vi "Get Python Version from Venv.vi"(8 "error in":errorcluster, 11 "venv":path) -> (0 "error out":errorcluster, 3 "Python Version":string)   [LabVIEW 2026]
doc: "Gets the Python version from a virtual-environment root path. Validates the input path and allowed characters, verifies that the expected Python executable exists, runs the interpreter with --version, and returns the parsed major.minor.patch version string. Returns an error if the venv path is invalid or the Python executable is missing."
uses:
  <vilib>/regexp/Match Regular Expression.xnode
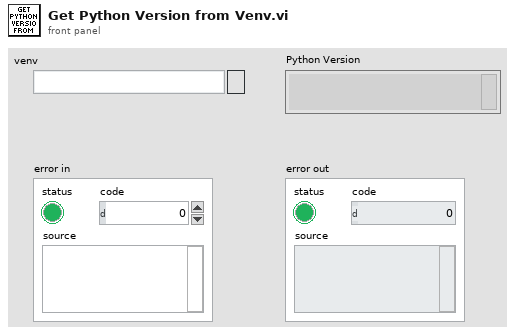
[diagram p1: front panel]
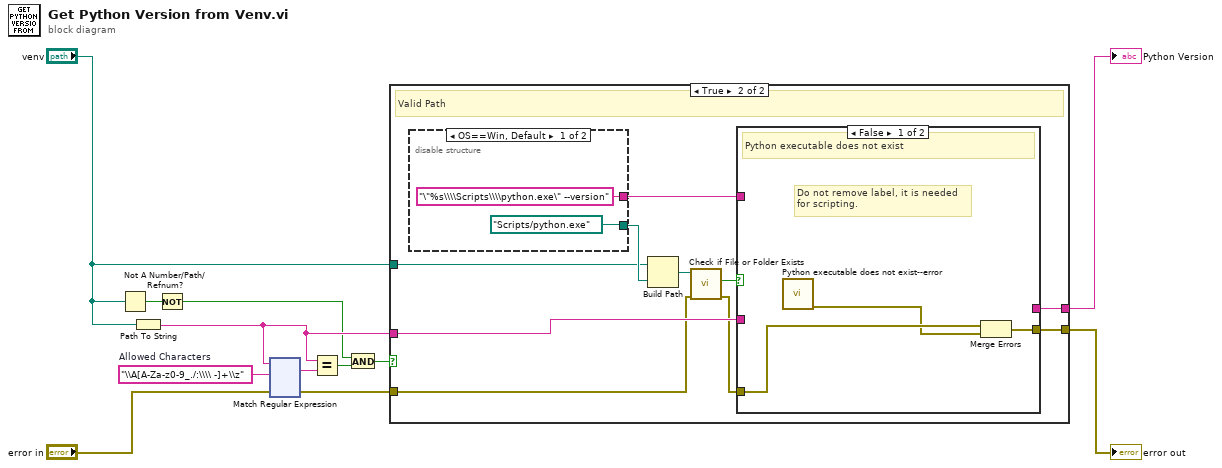
[diagram p0: block diagram]
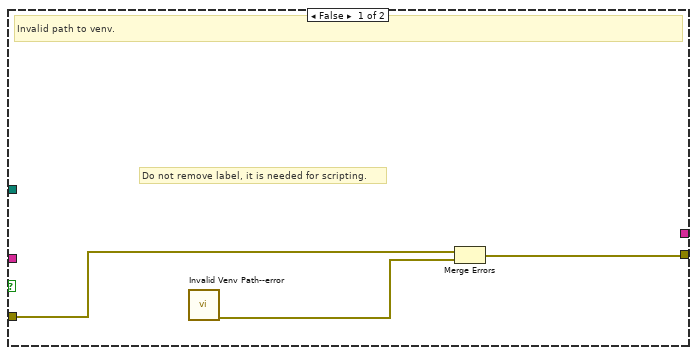
[diagram p2: hidden frame]
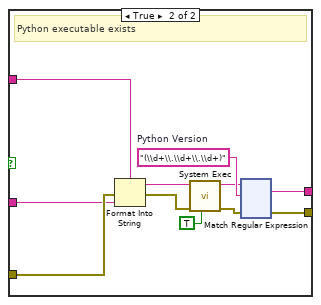
[diagram p3: hidden frame]
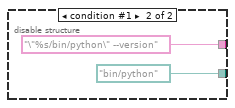
[diagram p4: hidden frame]
diagram:
  w7 = "\\A[A-Za-z0-9_./:\\\\ -]+\\z"  # Allowed Characters
  n1 = Not A Number/Path/Refnum?(number/path/refnum="venv") -> (NaN/Path/Refnum?=w2:bool)
  n2 = Path To String(path="venv") -> (string=w4:string)
  n3 = Not(x=w2) -> (.not. x?=w1:bool)
  n4 = xnode "Match Regular Expression"("input string"=w4, "regular expression"=w7, "error in"="error in") -> ("whole match"=w8:string, "error out"=w10:errorcluster)  [unwired: 3 in, 3 out]
  n5 = Equal?(x=w4, y=w8) -> (x = y?=w6:bool)
  n6 = And(x=w1, y=w6) -> (x .and. y?=w5:bool)
  n7 = case shown="True" w5 {
    tunnel: w10 -> [w15 w17]
    tunnel: [w14 w25] -> w12
    tunnel: [_ w23] -> w9
    tunnel: "venv" -> [_ w21]
    tunnel: w4 -> [_ w20]
    frame False {
      # "Do not remove label, it is needed for scripting."
      # "Invalid path to venv."
      n8 = call "Invalid Venv Path--error.vi"() -> ("error out"=w13:errorcluster)  [unwired: 11 in]
      n9 = Merge Errors(w15, w13) -> (w14:errorcluster)
    }
    frame True {
      # "Valid Path"
      n10 = disable-structure shown="OS==Win, Default" {
        disable-tunnel: ["\"%s\\\\Scripts\\\\python.exe\" --version" ("format string") "\"%s/bin/python\" --version" ("format string")] -> w24
        disable-tunnel: [path "Scripts/python.exe" path "bin/python"] -> w22
        frame condition #0 (active) {
        }
        frame condition #1 {
        }
      }
      n11 = Build Path(base path=w21, name or relative path=w22) -> (appended path=w19:path)
      n12 = call <vilib>:"Check if File or Folder Exists.vi"("error in (no error)"=w17, "path"=w19) -> ("error out"=w18:errorcluster, "file or folder exists?"=w16:bool)  [unwired: 7 in, 1 out]
      n13 = case shown="False" w16 {
        tunnel: w18 -> [w28 w38]
        tunnel: [w26 w36] -> w25
        tunnel: w24 -> [_ w35]
        tunnel: w20 -> [_ w34]
        tunnel: [_ w29] -> w23
        frame False {
          # "Do not remove label, it is needed\nfor scripting."
          # "Python executable does not exist"
          n14 = call "Python executable does not exist--error.vi"() -> ("error out"=w27:errorcluster)  [unwired: 11 in]
          n15 = Merge Errors(w28, w27) -> (w26:errorcluster)
        }
        frame True {
          w31 = "(\\d+\\.\\d+\\.\\d+)"  # Python Version
          # "Python executable exists"
          n16 = Format Into String(format string=w35, error in=w38, w34) -> (resulting string=w33:string, error out=w39:errorcluster)  [unwired: 1 in]
          n17 = call <vilib>:"System Exec.vi"("run minimized? (F)"=TRUE, "error in (no error)"=w39, "command line"=w33) -> ("error out"=w37:errorcluster, "standard output"=w30:string)  [unwired: 5 in, 2 out]
          n18 = xnode "Match Regular Expression"("input string"=w30, "regular expression"=w31, "error in"=w37) -> ("whole match"=w29:string, "error out"=w36:errorcluster)  [unwired: 3 in, 3 out]
        }
      }
    }
  }
  "error out" <- w12
  "Python Version" <- w9
